vi "Untitled 3.vi"() -> ()   [LabVIEW 2026, in "My Cloneable Module.lvlib"]
uses:
  My Cloneable Module.lvlib
panel:
  out "error out 2":errorcluster
  in  "Module ID 2":i32=-1
  in  "Error":errorcluster
  in  "Additional Information":string
  in  "error in 2":errorcluster
  out "error out":errorcluster
  in  "Module ID":i32=-1
  in  "Do Something Message":string
  in  "error in":errorcluster
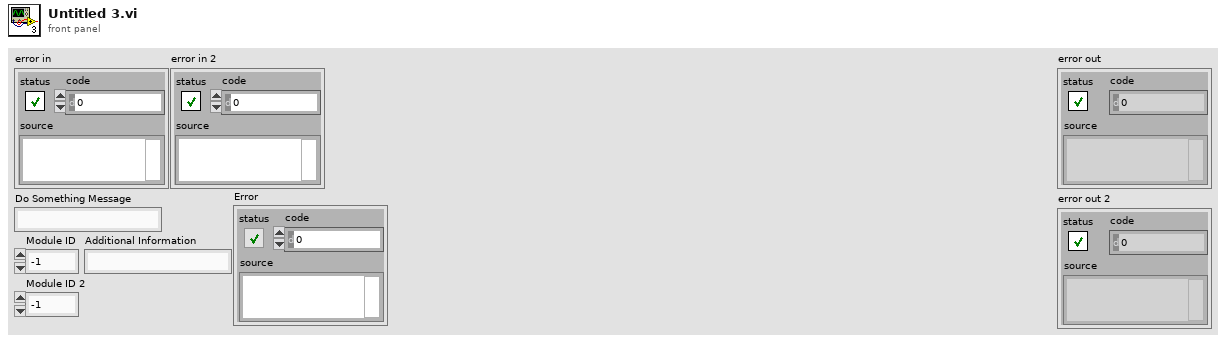
[diagram p1: front panel]
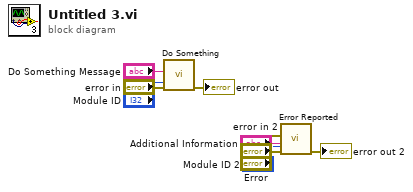
[diagram p0: block diagram]
diagram:
  n1 = call "Do Something.vi"("error in"="error in", "Do Something Message"="Do Something Message", "Module ID"="Module ID") -> ("error out"=→"error out":errorcluster)  [unwired: 8 in]
  n2 = call "Error Reported.vi"("error in"="error in 2", "Additional Information"="Additional Information", "Error"="Error", "Module ID"="Module ID 2") -> ("error out"=→"error out 2":errorcluster)  [unwired: 7 in]
